vi "LinearFilter_New.vi"(9 "OutputGains":dbl[](array[numeric]) format="%13.5p", 11 "InputGains":dbl[](array[numeric]) format="%13.5p") -> (3 "LINEAR_FILTER":T1 {"Outputs" format="%13.5g"; "Inputs" format="%13.5g"; "OutputGains" format="%13.5g"; "InputGains" format="%13.5g"})   [LabVIEW 2019, in "Trajectory_Library.lvlib"]
doc: "This VI creates a new data structure (cluster) that stores the data for a set of Vis that implement a linear, digital filter. All types of FIR and IIR filters are supported. A set of VIs are provided to create commonly used types of filters.\n \nFilters are of the form: \n y[n] = (b0*x[n] + b1*x[n-1] + ... + bP*x[n-P]) - (a0*y[n-1] + a2*y[n-2] + ... + aQ*y[n-Q])\n \nWhere: \ny[n] is the output at time \"n\" \nx[n] is the input at time \"n\" \ny[n-1] is the output from the LAST time step (\"n-1\") \nx[n-1] is the input from the LAST time step (\"n-1\") \nb0...bP are the \"feedforward\" (FIR) gains \na0...aQ are the \"feedback\" (IIR) gains \n\nIMPORTANT! Note the \"-\" sign in front of the feedback term! This is a common convention in signal processing.\n \nWhat can linear filters do? Basically, they can filter, or diminish, the effects of undesirable input frequencies. High frequencies, or rapid changes, can be indicative of sensor noise or be otherwise undesirable. A \"low pass\" filter smooths out the signal, reducing the impact of these high frequency components. Likewise, a \"high pass\" filter gets rid of slow-moving signal components, letting you detect large changes more easily.\n \nExample FRC applications of filters: \n- Getting rid of noise from an analog sensor input (note: the roboRIO's FPGA can do this faster in hardware)\n- Smoothing out joystick input to prevent the wheels from slipping or the robot from tipping\n- Smoothing motor commands so that unnecessary strain isn't put on electrical or mechanical components\n- If you use clever gains, you can make a PID controller out of this class! (Use the PID set of VI’s instead...)\n \nFor more on filters, we highly recommend the following articles:\n https://en.wikipedia.org/wiki/Linear_filter\n https://en.wikipedia.org/wiki/Iir_filter\n https://en.wikipedia.org/wiki/Fir_filter\n \nNote 1: calculate() should be called by the user on a known, regular period. You can use code in a periodic function.\n \nNote 2: For ALL filters, gains are necessarily a function of frequency. If you make a filter that works well for you at, say, 100Hz, (executing every 10 milliseconds ), you will most definitely need to adjust the gains if you then want to run it at 200Hz, (executing every 5 milliseconds)! Combining this with Note 1, the impetus is on YOU as a developer to make sure calculate() gets called at the desired, constant frequency!\n\nInputs: \n - InputGains - Array of “feedforward” or FIR gain factors (bx)\n\n - OutputGains - Array of “feedback” or IIR gain factors for feedback terms (ax)\n\nOutputs:\n - LINEAR FILTER - cluster containing:\n - InputGains - Array of “feedforward” or FIR gain factors (bx)\n - OutputGains - Array of “feedback” or IIR gain factors for feedback terms (ax)\n - Inputs - Array of the last n saved inputs\n - Outputs - Array of the last n saved outputs\n - InGainCount - Number of input gain terms\n - OutGainCount - number of output gain terms"
uses:
  Trajectory_Library.lvlib
  TypeDef/LINEAR_FILTER.ctl
  <vilib>/Rock Robotics/SystemInterfaces/NetworkCommunication/NetComm_UsageReport_ResourceType.ctl
  Globals/Util_LibraryGlobals.vi
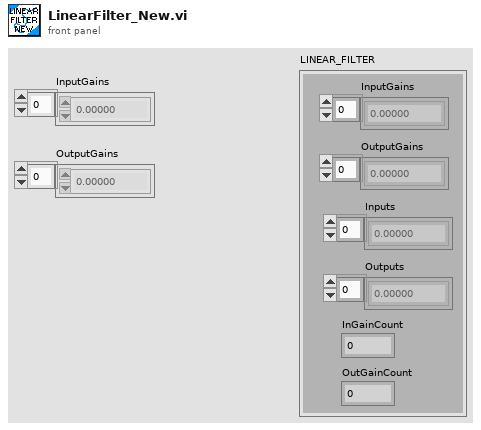
[diagram p1: front panel]
types:
  T1 = typedef "Trajectory_Library.lvlib/LINEAR_FILTER.ctl" = cluster{"InputGains":dbl[], "OutputGains":dbl[], "Inputs":dbl[], "Outputs":dbl[], "InGainCount":i32, "OutGainCount":i32}
  T2 = typedef "NetComm_UsageReport_ResourceType.ctl" = enum8{"Controller", "Module", "Language", "CANPlugin", "Accelerometer", "ADXL345", "AnalogChannel", "AnalogTrigger", "AnalogTriggerOutput", "CANJaguar", "Compressor", "Counter", "Dashboard", "DigitalInput", "DigitalOutput", "DriverStationCIO", "DriverStationEIO", "DriverStationLCD", "Encoder", "GearTooth", "Gyro", "I2C", "Framework", "Jaguar", "Joystick", "Kinect", "KinectStick", "PIDController", "Preferences", "PWM", "Relay", "RobotDrive", "SerialPort", "Servo", "Solenoid", "SPI", "Task", "Ultrasonic", "Victor", "Button", "Command", "AxisCamera", "PCVideoServer", "SmartDashboard", "Talon", "HiTechnicColorSensor", "HiTechnicAccel", "HiTechnicCompass", "SRF08", "AnalogOutput", "Victor SP", "Talon SRX", "CAN Talon SRX", "ADXL362 Accel", "ADXRS450 Gyro", "Rev SPARK", "Mindsensors SD540", "Digital Filter", "ADIS16448", "PDP", "PCM", "PigeonIMU", "Nidec Brushless", "CTRE CANifier", "CTRE TalonFX", "CTRE Future 1", "CTRE Future 2", "CTRE Future 3", "CTRE Future 4", "CTRE Future 5", "CTRE Future 6", "Linear Filter", "Xbox Controller", "USB Camera", "NavX", "Pixy", "Pixy2", "ScanseSweep", "Shuffleboard", "CAN", "Digilent DMC60", "PWM Victor SPX", "Rev SPARK MAX PWM", "Rev SPARK MAX CAN", "ADIS16470", "PIDController2", "ProfiledPIDController", "Kinematics", "Odometry", "Units", "Trapezoid Profile", "DutyCycle", "Addressable LEDs", "Fusion Venom"}
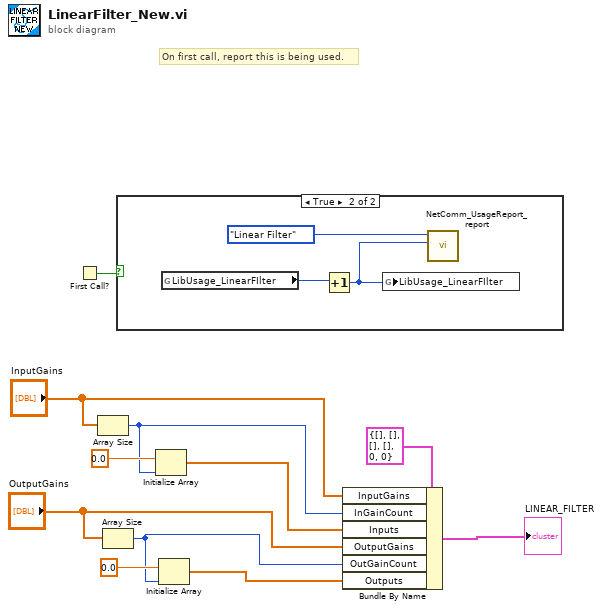
[diagram p0: block diagram]
diagram:
  # "On first call, report this is being used."
  n1 = First Call?() -> (First Call?: T/F=w1:bool)
  n2 = Array Size(array="InputGains") -> (size(s)=w6:i32)
  n3 = Array Size(array="OutputGains") -> (size(s)=w3:i32)
  n4 = case shown="True" w1 {
    frame False {
    }
    frame True {
      n5 = global read "Util_LibraryGlobals.vi" "LibUsage_LinearFIlter"() -> (w13:i32)
      n6 = Increment(x=w13) -> (x+1=w12:i32)
      n7 = global write "Util_LibraryGlobals.vi" "LibUsage_LinearFIlter"(w12) -> ()
      n8 = call <vilib>:"NetComm_UsageReport_report.vi"("Instance Number"=w12, "Resource Type"=NetComm_UsageReport_ResourceType."Linear Filter") -> ()  [unwired: 10 in]
    }
  }
  n9 = Initialize Array(0.0, w6) -> (w5:dbl[])
  n10 = Initialize Array(0.0, w3) -> (w2:dbl[])
  n11 = Bundle By Name(cluster=T1 {"InputGains"=[], "OutputGains"=[], "Inputs"=[], "Outputs"=[], "InGainCount"=0, "OutGainCount"=0} ("LINEAR_FILTER"), "InputGains"="InputGains", "InGainCount"=w6, "Inputs"=w5, "OutputGains"="OutputGains", "OutGainCount"=w3, "Outputs"=w2) -> (→"LINEAR_FILTER":T1)
